vi "Prepare Response.vi"(8 "error in (no error)":errorcluster, 11 "PUBREL in":refnum<class "PUBREL.lvclass">) -> (0 "error out":errorcluster, 1 "response prepared?":bool, 2 "ControlPacket response":refnum<class "ControlPacket.lvclass">, 3 "PUBREL out":refnum<class "PUBREL.lvclass">)   [LabVIEW 2013, in "MQTT_Control_Packets.lvlib" / "PUBREL.lvclass"]
uses:
  PUBREL.lvclass
  ControlPacket/ControlPacket.lvclass
  ControlPacket/ControlPacket.lvclass/ControlPacket.ctl
  PUBCOMP/PUBCOMP.lvclass
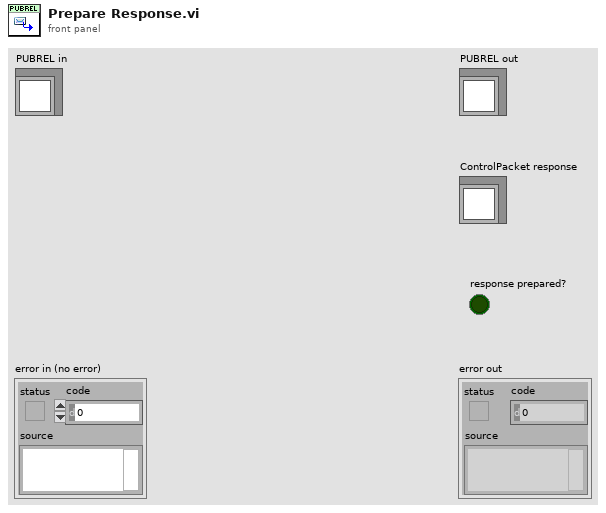
[diagram p1: front panel]
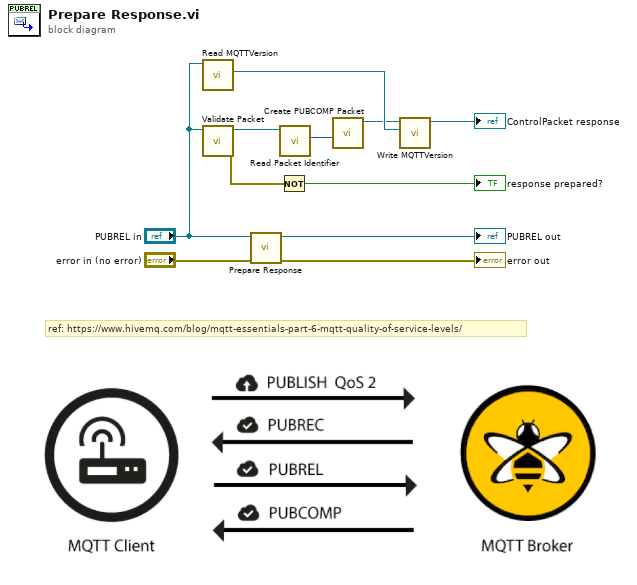
[diagram p0: block diagram]
diagram:
  # "ref: https://www.hivemq.com/blog/mqtt-essentials-part-6-mqtt-quality-of-service-levels/"
  n1 = call "Read MQTTVersion.vi"("ControlPacket in"="PUBREL in") -> ("MQTTVersion"=w3:refnum<class "MQTTVersion.lvclass">)  [unwired: 9 in, 1 out]
  n2 = call "Validate Packet.vi"("ControlPacket in"="PUBREL in") -> ("error out"=w7:errorcluster, "ControlPacket out"=w8:refnum<class "PUBREL.lvclass">)  [unwired: 9 in]
  n3 = call-parent "Prepare Response.vi"("error in (no error)"="error in (no error)", "ControlPacket in"="PUBREL in") -> ("error out"=→"error out":errorcluster, "ControlPacket out"=→"PUBREL out":refnum<class "PUBREL.lvclass">)  [unwired: 6 in, 2 out]
  n4 = Not(x=w7) -> (.not. x?=→"response prepared?":bool)
  n5 = call "Read Packet Identifier.vi"("ControlPacket in"=w8) -> ("Packet Identifier"=w6:u16)  [unwired: 9 in, 1 out]
  n6 = call "Create PUBCOMP Packet.vi"("Packet ID"=w6) -> ("PUBCOMP out"=w2:refnum<class "PUBCOMP.lvclass">)  [unwired: 8 in, 2 out]
  n7 = call "Write MQTTVersion.vi"("MQTTVersion"=w3, "ControlPacket in"=w2) -> ("ControlPacket out"=→"ControlPacket response":refnum<class "PUBCOMP.lvclass">)  [unwired: 9 in]
